vi "Read Test Manager.vi"(8 "error in (no error)":errorcluster, 10 "VI Call Chain":string[](array[string]), 11 "Assert Factory in":refnum<class "Test Assert Factory.lvclass">) -> (0 "error out":errorcluster, 2 "Basic Test Manager":refnum<class "Basic Test Manager.lvclass">, 3 "Assert Factory out":refnum<class "Test Assert Factory.lvclass">)   [LabVIEW 2013, in "Caraya.lvlib" / "Test Assert Factory.lvclass"]
doc: "Returns the Test Manager implementation being used for a specific VI."
uses:
  Test Assert Factory.lvclass
  Basic Test Manager/Basic Test Manager.lvclass
  Test Assert Factory.lvclass/Test Assert Factory.ctl
  Basic Test Manager/Basic Test Manager.lvclass/Basic Test Manager.ctl
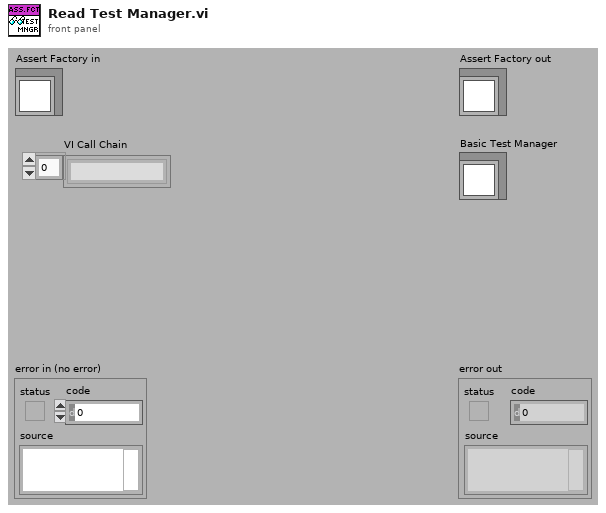
[diagram p1: front panel]
types:
  T1 = typedef "Caraya.lvlib/Test Result.lvclass/Test Events -- cluster.ctl" = cluster{"Test Registration Event":refnum<user-event>, "Assertion Event":refnum<user-event>, "Assertion Update Event":refnum<user-event>}
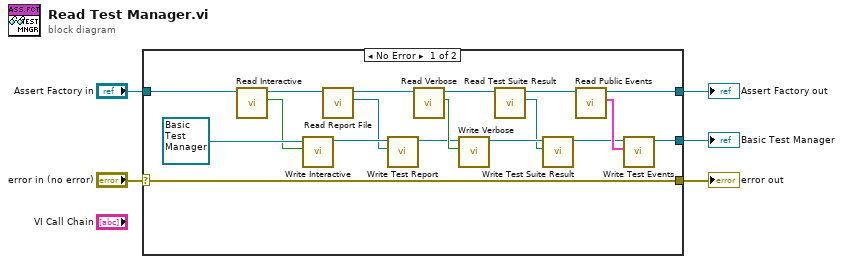
[diagram p0: block diagram]
diagram:
  n1 = case shown="No Error" "error in (no error)" {
    selector: "error in (no error)" -> [w6 w25]
    tunnel: "Assert Factory in" -> [w22 w24]
    tunnel: [w12 w24] -> w4
    tunnel: [w9 _] -> w3
    tunnel: [w6 w25] -> w2
    frame No Error {
      n2 = call "Read Interactive.vi"("Test Assert Factory in"=w22) -> ("Interactive"=w21:bool, "Test Assert Factory out"=w20:refnum<class "Test Assert Factory.lvclass">)  [unwired: 8 in, 1 out]
      n3 = call "Write Interactive.vi"("Interactive"=w21, "Basic Test Manager in"=refnum<class "Basic Test Manager.lvclass"> refnum ("Caraya.lvlib:Basic Test Manager.lvclass")) -> ("Basic Test Manager out"=w19:refnum<class "Basic Test Manager.lvclass">)  [unwired: 8 in, 1 out]
      n4 = call "Read Report File.vi"("Test Assert Factory in"=w20) -> ("Test Report"=w18:refnum<class "Test Report.lvclass">, "Test Assert Factory out"=w7:refnum<class "Test Assert Factory.lvclass">)  [unwired: 8 in, 1 out]
      n5 = call "Write Test Report.vi"("Test Report"=w18, "Basic Test Manager"=w19) -> ("Basic Test Manager"=w8:refnum<class "Basic Test Manager.lvclass">)  [unwired: 9 in]
      n6 = call "Read Verbose.vi"("Test Assert Factory in"=w7) -> ("Verbose"=w17:bool, "Test Assert Factory out"=w16:refnum<class "Test Assert Factory.lvclass">)  [unwired: 8 in, 1 out]
      n7 = call "Write Verbose.vi"("Verbose"=w17, "Basic Test Manager"=w8) -> ("Basic Test Manager"=w15:refnum<class "Basic Test Manager.lvclass">)  [unwired: 8 in, 1 out]
      n8 = call "Read Test Suite Result.vi"("Test Assert Factory in"=w16) -> ("Test Suite Result"=w14:refnum<user-event>, "Test Assert Factory out"=w13:refnum<class "Test Assert Factory.lvclass">)  [unwired: 8 in, 1 out]
      n9 = call "Write Test Suite Result.vi"("Test Suite Result"=w14, "Basic Test Manager in"=w15) -> ("Basic Test Manager out"=w10:refnum<class "Basic Test Manager.lvclass">)  [unwired: 8 in, 1 out]
      n10 = call "Read Public Events.vi"("Test Assert Factory in"=w13) -> ("Public Events"=w11:T1, "Test Assert Factory out"=w12:refnum<class "Test Assert Factory.lvclass">)  [unwired: 8 in, 1 out]
      n11 = call "Write Test Events.vi"("Test Events"=w11, "Basic Test Manager in"=w10) -> ("Basic Test Manager out"=w9:refnum<class "Basic Test Manager.lvclass">)  [unwired: 8 in, 1 out]
    }
    frame Error {
    }
  }
  "error out" <- w2
  "Assert Factory out" <- w4
  "Basic Test Manager" <- w3
